vi "Port To Labels.vi"(8 "error in":errorcluster, 11 "port ref":T6 format="%.0x") -> (0 "error out":errorcluster, 2 "labels":T1[](array[typedef]), 3 "port ref out":T6 format="%.0x")   [LabVIEW 2020, in "AIM ARINC 429 Scripting.lvlib"]
uses:
  AIM ARINC 429 Scripting.lvlib
  <vilib>/NI VeriStand/Custom Device API/Custom Device Item Ref.ctl
  Shared/VS Channels Definition for Label.ctl
  Shared/VS Channel Definition for Parameter.ctl
  Shared/Parameter Definition.ctl
  <vilib>/NI/NI VeriStand Encoding and Decoding/Encoding.ctl
  Shared/Transfer Type.ctl
  <vilib>/NI/NI VeriStand Encoding and Decoding/Encoding and Decoding.lvlib
  <vilib>/NI VeriStand/Custom Device API/Custom Device API.lvlib
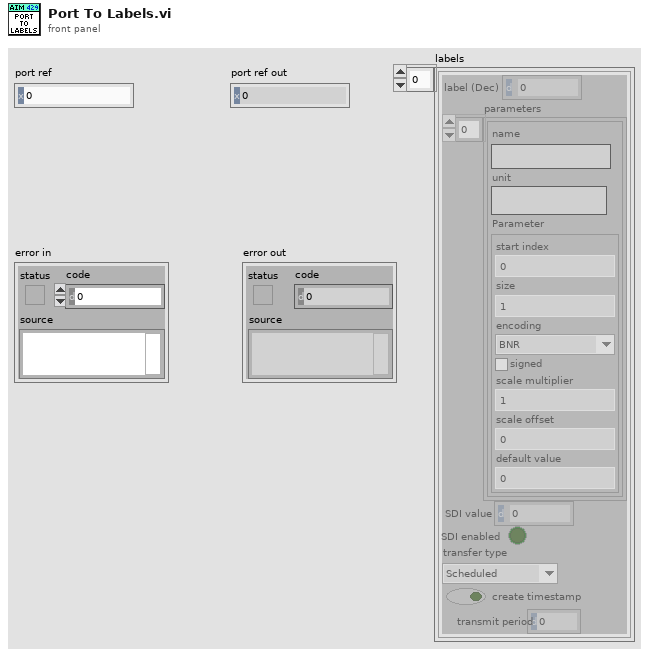
[diagram p1: front panel]
types:
  T1 = typedef "VS Channels Definition for Label.ctl" = cluster{"label (Dec)":u32, "parameters":T2[], "SDI value":u8, "SDI enabled":bool, "transfer type":T5, "create timestamp":bool, "transmit period":u32}
  T2 = typedef "VS Channel Definition for Parameter.ctl" = cluster{"name":string, "unit":string, "Parameter":T3}
  T3 = typedef "Parameter Definition.ctl" = cluster{"start index":i32, "size":i32, "encoding":T4, "signed":bool, "scale multiplier":dbl, "scale offset":dbl, "default value":dbl}
  T4 = typedef "Encoding and Decoding.lvlib/Encoding.ctl" = enum16{"BNR", "BCD", "Discrete"}
  T5 = typedef "Transfer Type.ctl" = enum16{"Scheduled", "Acyclic", "Block", "Strobe"}
  T6 = typedef "Custom Device API.lvlib/Custom Device Item Ref.ctl" = u64
  T7 = typedef "Label Properties.ctl" = cluster{"label (Dec)":T8, "SDI value":u8, "SDI enabled":bool}
  T8 = typedef "Label.ctl" = u8
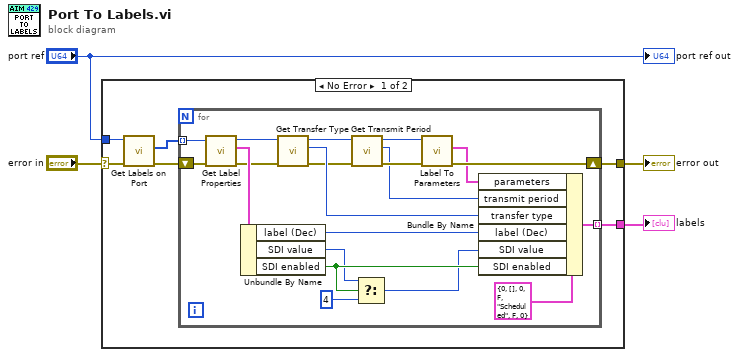
[diagram p0: block diagram]
diagram:
  n1 = case shown="No Error" "error in" {
    selector: "error in" -> [w5 w31]
    tunnel: "port ref" -> [w6 _]
    tunnel: [w9 w31] -> w4
    tunnel: [w10 _] -> w1
    frame No Error {
      n2 = call "Get Labels on Port.vi"("error in"=w5, "port ref"=w6) -> ("error out"=w8:errorcluster, "labels"=w7:T6[])  [unwired: 6 in, 2 out]
      n3 = for {
        tunnel: w7 -> [w29] mode=indexing
        tunnel: [w17] -> w10 mode=indexing
        shift-right: [w18] -> w9
        shift-left: w8 -> [w30]
        n4 = call "Get Label Properties.vi"("error in"=w30, "label ref"=w29) -> ("error out"=w26:errorcluster, "label properties"=w27:T7, "label ref out"=w25:T6)  [unwired: 6 in, 1 out]
        n5 = Unbundle By Name(w27) -> ("label (Dec)"=w23:T8, "SDI value"=w21:u8, "SDI enabled"=w22:bool)
        n6 = call "Get Transfer Type.vi"("error in"=w26, "label ref"=w25) -> ("error out"=w16:errorcluster, "transfer type"=w24:T5, "label ref out"=w15:T6)  [unwired: 7 in]
        n7 = call "Get Transmit Period.vi"("error in"=w16, "label ref"=w15) -> ("error out"=w13:errorcluster, "transmit period (us)"=w11:u32, "label ref out"=w14:T6)  [unwired: 7 in]
        n8 = Select(t=w21, s=w22, f=u8 4 ("SDI value")) -> (s? t:f=w19:u8)
        n9 = call "Label To Parameters.vi"("error in"=w13, "label ref"=w14) -> ("error out"=w18:errorcluster, "parameters"=w12:T2[])  [unwired: 7 in, 1 out]
        n10 = Bundle By Name(cluster=T1 {"label (Dec)"=0, "parameters"=[], "SDI value"=0, "SDI enabled"=FALSE, "transfer type"=enum."Scheduled", "create timestamp"=FALSE, "transmit period"=0} ("label parameters"), "parameters"=w12, "transmit period"=w11, "transfer type"=w24, "label (Dec)"=w23, "SDI value"=w19, "SDI enabled"=w22) -> (w17:T1)
      }
    }
    frame Error {
    }
  }
  "error out" <- w4
  "labels" <- w1
  "port ref out" <- "port ref"
